vi "Add Text.vi"(8 "error in (no error)":errorcluster, 10 "text":string, 11 "reference":refnum<k24>) -> (0 "error out":errorcluster, 3 "reference out":refnum<k24>)   [LabVIEW 2026, in "ToastNotification.lvlib" / "Toast Native.lvlib"]
doc: "Native AddText call. Append displayed text to a borrowed ToastContentBuilder and return the builder alias. Does not create an activation argument, show the toast or close the handle."
uses:
  Toast Native.lvlib
  C:/Users/loicw/Documents/LabVIEW/ToastNotifications/Sources/bins/Microsoft.Toolkit.Uwp.Notifications.dll
  bins/Microsoft.Toolkit.Uwp.Notifications.dll
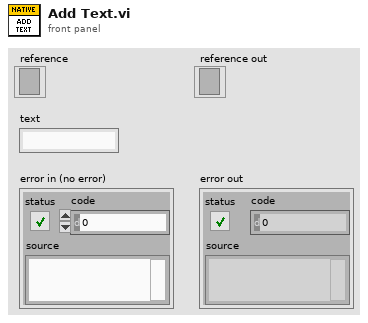
[diagram p1: front panel]
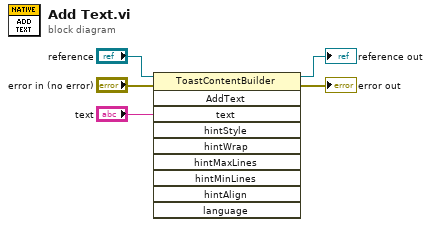
[diagram p0: block diagram]
diagram:
  n1 = invoke class="ToastContentBuilder" method="AddText"(reference="reference", error in="error in (no error)", "text"="text") -> (reference out=→"reference out":refnum<k24>, error out=→"error out":errorcluster)  [unwired: 7 in, 8 out]
